vi "FuncVI-Median.vi"(5 "InstanceRef":T2, 9 "arg list":T1[](array[typedef]) {"num" format="%.2f"}) -> (0 "error out":bool, 3 "result":T1 {"num" format="%.2f"})   [LabVIEW 2021]
doc: "::: CalcExpress Toolkit :::\nCopyright (c) 2000-2026 Konstantin Shifershteyn. All rights reserved."
uses:
  cetypes.llb/CalcExpress Function Argument Info.ctl
  cetypes.llb/CalcExpress Instance RefNum.ctl
  <vilib>/Analysis/NI_AALBase.lvlib
panel:
  in  "max arg num":i32=1
  in  "min arg num":i32=1
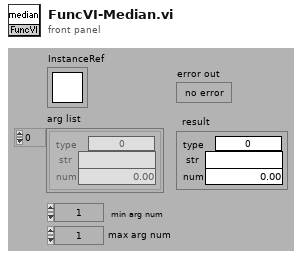
[diagram p1: front panel]
types:
  T1 = typedef "CalcExpress Function Argument Info.ctl" = cluster{"type":u32, "str":string, "num":dbl}
  T2 = typedef "CalcExpress Instance RefNum.ctl" = refnum<k1>
  T3 = enum32{"String", "DBL Number", "identifier", "1D Array of DBL", "2D Array of DBL", "CDB Number", "1D Array of CDB", "2D Array of CDB", "1D Array of String", "2D Array of String", "Unknown data type"}
  T4 = cluster{"use this constant to specify a predefined type":enum32{"String", "DBL Number", "identifier", "1D Array of DBL", "2D Array of DBL", "CDB Number", "1D Array of CDB", "2D Array of CDB", "1D Array of String", "2D Array of String", "Unknown data type"}, string, "median":dbl}
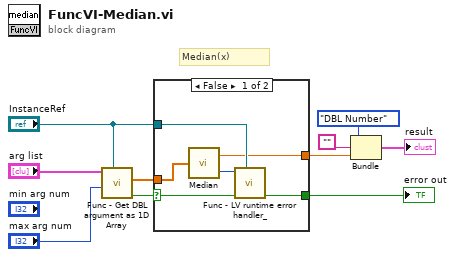
[diagram p0: block diagram]
diagram:
  # "Median(x)"
  n1 = call "Func - Get DBL argument as 1D Array.vi"("InstanceRef"="InstanceRef", "max arg num"="max arg num", "arg list"="arg list") -> ("error out"=w10:bool, "1D data"=w9:dbl[])  [unwired: 5 in, 2 out]
  n2 = case shown="False" w10 {
    selector: w10 -> [w15 w17]
    tunnel: w9 -> [w16 _]
    tunnel: [w11 _] -> w5
    tunnel: [w13 w17] -> w6
    tunnel: "InstanceRef" -> [w12 _]
    frame False {
      n3 = call <vilib>:"Median.vi"("X"=w16) -> ("median"=w11:dbl, "error"=w14:i32)
      n4 = call "Func - LV runtime error handler_.vi"("InstanceRef"=w12, "error in"=w15, "LabVIEW error code"=w14) -> ("error out"=w13:bool)  [unwired: 8 in]
    }
    frame True {
    }
  }
  "error out" <- w6
  n5 = Bundle("use this constant to specify a predefined type"=T3."DBL Number", "", "median"=w5) -> (→"result":T4)  [unwired: 1 in]
